vi "PicoScope5000aSetupStreaming.vi"(0 "error in":errorcluster, 1 "Device Info":T2, 2 "handle in":i16, 3 "Acquisition Settings":T3={"Auto Stop"=FALSE, "Desired Sample Interval"=4, "Pre-trigger Samples"=0, "Post-trigger Samples"=1000, "Down-Sample Ratio"=1, "Down-Sample Mode"=0, "Time Units"=2} {"Time Units" items=["Nanoseconds (ns)"=2, "Microseconds (us)"=3, "Milliseconds (ms)"=4, "Seconds (s)"=5]; "Down-Sample Mode" items=["None"=0, "Aggregate"=1, "Decimate"=2, "Average"=4]}, 4 "Buffer and Transfer Settings":T1={"startIndex"=0, "Samples"=1000000, "Down Sample Ratio"=1, "Down-Sample Mode"=0} {"Down-Sample Mode" items=["None"=0, "Aggregate"=1, "Decimate"=2, "Average"=4]; "Down Sample Ratio" step=1; "Samples" format="%_6p"}, 5 "enabled array":i16[](array[numeric]), 10 "Pointers In":u64[][](array[numeric])) -> (11 "Pointer array":u64[][](array[numeric]), 14 "error out":errorcluster, 16 "handle out":i16, 17 "Sample Interval":u32, 19 "sampleIntervalTimeUnits":u32)   [LabVIEW 2010]
doc: "Set up the data buffers and calls RunStreaming to start the device streaming.\nData will be copied from the driver buffers into the corresponding application buffers using the wrapper dll."
uses:
  ps5000a.dll
  ps5000aWrap.dll
panel:
  # "Overview Buffer Size is the size of the temporary buffers used to\nstore data before returning it to the application."
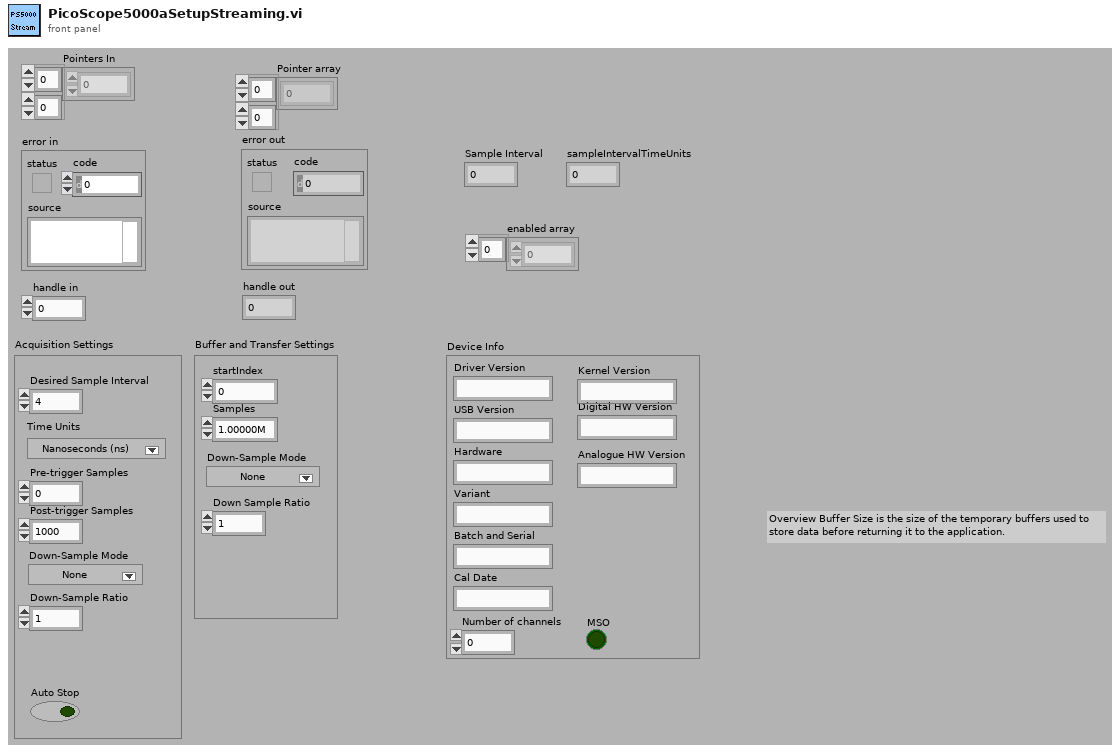
[diagram p1: front panel]
types:
  T1 = cluster{"startIndex":u64, "Samples":u64, "Down Sample Ratio":u64, "Down-Sample Mode":u32}
  T2 = cluster{"Driver Version":string, "USB Version":string, "Hardware":string, "Variant":string, "Batch and Serial":string, "Cal Date":string, "Kernel Version":string, "Digital HW Version":string, "Analogue HW Version":string, "MSO":bool, "Number of channels":i16}
  T3 = cluster{"Auto Stop":bool, "Desired Sample Interval":u32, "Pre-trigger Samples":u32, "Post-trigger Samples":u32, "Down-Sample Ratio":u32, "Down-Sample Mode":i32, "Time Units":u32}
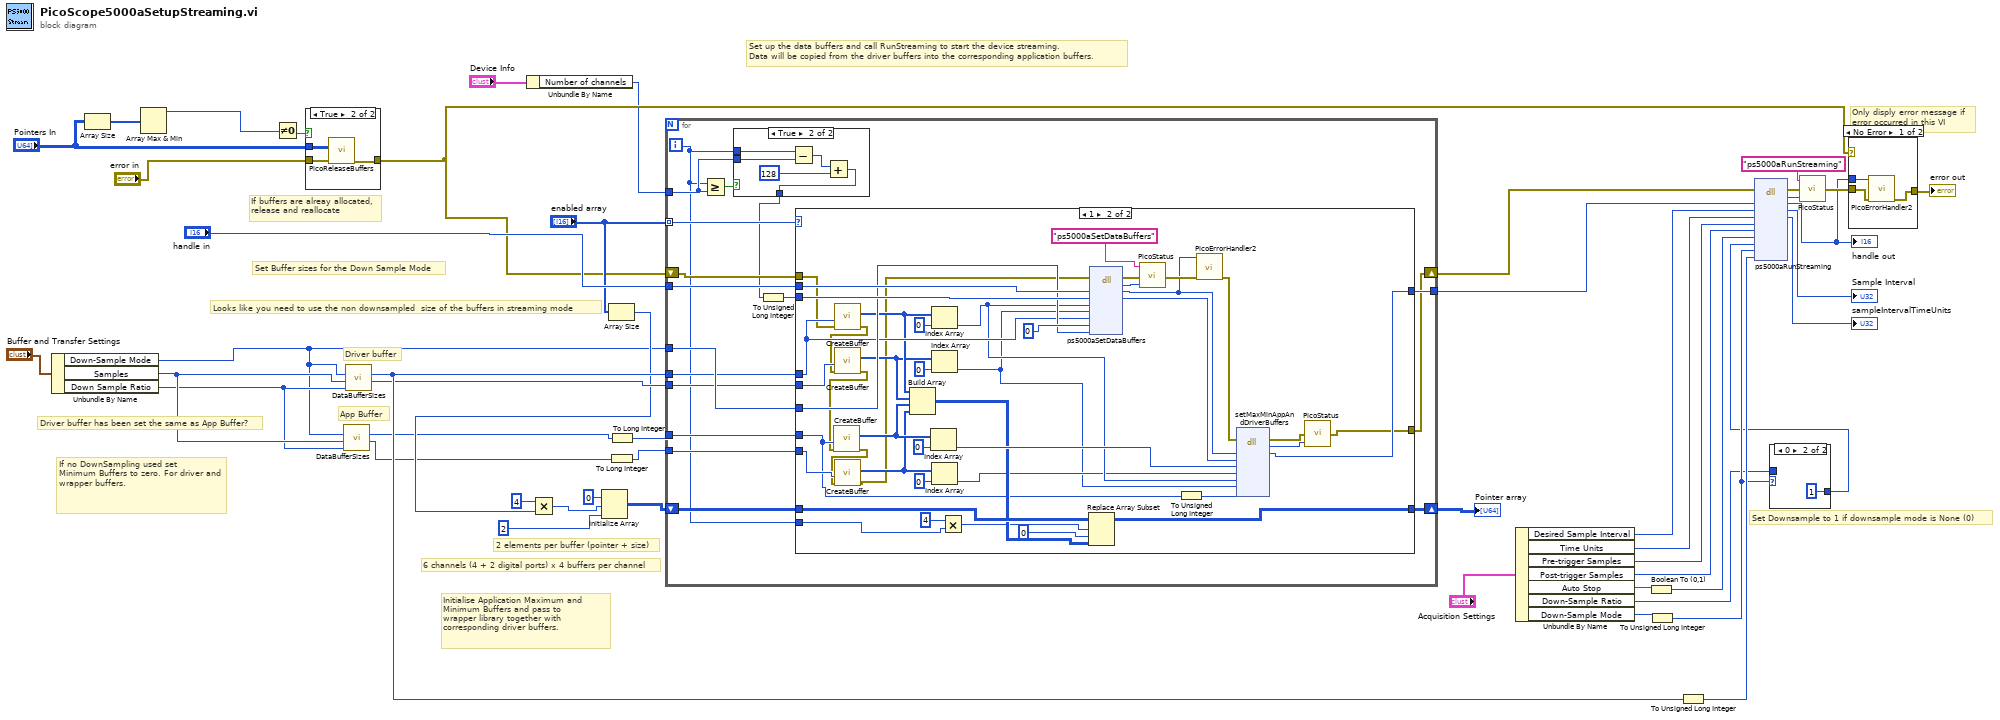
[diagram p0: block diagram]
diagram:
  # "Set Downsample to 1 if downsample mode is None (0)"
  # "Looks like you need to use the non downsampled  size of the buffers in streaming mode"
  # "If buffers are alreay allocated,\nrelease and reallocate"
  # "2 elements per buffer (pointer + size)"
  # "6 channels (4 + 2 digital ports) x 4 buffers per channel"
  # "App Buffer"
  # "Driver buffer"
  # "Driver buffer has been set the same as App Buffer?"
  # "Set Buffer sizes for the Down Sample Mode"
  # "If no DownSampling used set \nMinimum Buffers to zero. For driver and wrapper buffers."
  # "Initialise Application Maximum and\nMinimum Buffers and pass to \nwrapper library together with corresponding driver buffers."
  # "Only disply error message if\nerror occurred in this VI"
  # "Set up the data buffers and call RunStreaming to start the device streaming.\nData will be copied from the driver buffers into the corresponding application buffers."
  n1 = Unbundle By Name("Buffer and Transfer Settings") -> ("Down-Sample Mode"=w9:u32, "Samples"=w32:u64, "Down Sample Ratio"=w31:u64)
  n2 = Array Size(array="Pointers In") -> (size(s)=w12:i32[])
  n3 = Array Max & Min(array=w12) -> (max value=w11:i32)  [unwired: 3 out]
  n4 = Not Equal To 0?(x=w11) -> (x != 0?=w18:bool)
  n5 = case shown="True" w18 {
    tunnel: "Pointers In" -> [_ w51]
    tunnel: "error in" -> [w50 w52]
    tunnel: [w50 w53] -> w15
    frame False {
    }
    frame True {
      n6 = call "PicoReleaseBuffers.vi"("error in (no error)"=w52, "Pointer array"=w51) -> ("error out"=w53:errorcluster)  [unwired: 9 in]
    }
  }
  n7 = call "DataBufferSizes.vi"("Down Sample Ratio"=w31, "Number of Samples"=w32, "Down-Sample Mode"=w9) -> ("min Buffer Size"=w2:i32, "Max Buffer Size"=w3:i32)  [unwired: 7 in]
  n8 = call "DataBufferSizes.vi"("Down Sample Ratio"=w31, "Number of Samples"=w32, "Down-Sample Mode"=w9) -> ("min Buffer Size"=w29:i32, "Max Buffer Size"=w30:i32)  [unwired: 7 in]
  n9 = Unbundle By Name("Device Info") -> ("Number of channels"=w1:i16)
  n10 = Array Size(array="enabled array") -> (size(s)=w22:i32)
  n11 = Multiply(x=4, y=w22) -> (x*y=w23:i32)
  n12 = Initialize Array(u64 0 ("element"), w23, 2 ("dimension size")) -> (w13:u64[][])
  n13 = To Long Integer(number=w2) -> (32bit integer=w4:i32)
  n14 = To Long Integer(number=w3) -> (32bit integer=w5:i32)
  n15 = for {
    tunnel: "enabled array" -> [w62] mode=indexing
    tunnel: "handle in" -> [w70]
    tunnel: w9 -> [w69]
    tunnel: w5 -> [w68]
    tunnel: w30 -> [w67]
    tunnel: w29 -> [w66]
    tunnel: w4 -> [w65]
    tunnel: [w63] -> w25
    shift-right: [w61] -> w19
    shift-left: w15 -> [w60]
    shift-right: [w64] -> w28
    shift-left: w13 -> [w59]
    tunnel: w1 -> [w55]
    i -> [w54]
    n16 = Greater Or Equal?(x=w54, y=w55) -> (x >= y?=w57:bool)
    n17 = case shown="True" w57 {
      tunnel: [w71 w75] -> w56
      tunnel: w54 -> [w71 w73]
      tunnel: w55 -> [_ w72]
      frame False {
      }
      frame True {
        n18 = Subtract(x=w73, y=w72) -> (x-y=w74:i32)
        n19 = Add(x=w74, y=128) -> (x+y=w75:i32)
      }
    }
    n20 = To Unsigned Long Integer(number=w56) -> (unsigned 32bit integer=w58:u32)
    n21 = case shown="1" w62 {
      tunnel: w70 -> [w78 w123]
      tunnel: w60 -> [w77 w84]
      tunnel: w58 -> [_ w117]
      tunnel: w68 -> [_ w87]
      tunnel: w67 -> [_ w107]
      tunnel: w66 -> [_ w110]
      tunnel: w65 -> [_ w109]
      tunnel: w69 -> [_ w108]
      tunnel: w59 -> [w79 w101]
      tunnel: [w79 w100] -> w64
      tunnel: w54 -> [_ w97]
      tunnel: [w78 w93] -> w63
      tunnel: [w77 w92] -> w61
      frame 0, Default {
      }
      frame 1 {
        n22 = call "CreateBuffer.vi"("error in (no error)"=w84, "Buffer size"=w107) -> ("error out"=w83:errorcluster, "Pointer and BufferSize"=w105:u64[])  [unwired: 8 in]
        n23 = call "CreateBuffer.vi"("error in (no error)"=w83, "Buffer size"=w110) -> ("error out"=w82:errorcluster, "Pointer and BufferSize"=w104:u64[])  [unwired: 8 in]
        n24 = call "CreateBuffer.vi"("error in (no error)"=w82, "Buffer size"=w87) -> ("error out"=w81:errorcluster, "Pointer and BufferSize"=w103:u64[])  [unwired: 8 in]
        n25 = call "CreateBuffer.vi"("error in (no error)"=w81, "Buffer size"=w109) -> ("error out"=w80:errorcluster, "Pointer and BufferSize"=w102:u64[])  [unwired: 8 in]
        n26 = Build Array(w105, w104, w103, w102) -> (w96:u64[][])
        n27 = Index Array(array=w103, index=0) -> (element=w106:u64)
        n28 = Index Array(array=w105, index=0) -> (element=w99:u64)
        n29 = Index Array(array=w104, index=0) -> (element=w85:u64)
        n30 = Index Array(array=w102, index=0) -> (element=w86:u64)
        n31 = Multiply(x=4, y=w97) -> (x*y=w95:i32)
        n32 = Replace Array Subset(array=w101, new element=w96, index (row)=w95, index (col)=0 ("disabled index (row)")) -> (w100:u64[][])
        n33 = dll-call lib="ps5000a.dll" fn="ps5000aSetDataBuffers" ("ps3000.dll:_ps3000_open_unit@0")(error in=w80, "handle"=w123, "channel"=w117, "bufferMax"=w99, "bufferMin"=w85, "bufferLth"=w107, "segmentIndex"=u32 0, "downSampleRatioMode"=w108) -> (error out=w121:errorcluster, "PICO_STATUS"=w122:u32, "handle"=w89:i16, "channel"=w118:u32)  [unwired: 7 in, 1 out]
        n34 = call "PicoStatus.vi"("PICO STATUS"=w122, "error in"=w121, "source"="ps5000aSetDataBuffers") -> ("error out"=w91:errorcluster)
        n35 = To Unsigned Long Integer(number=w87) -> (unsigned 32bit integer=w88:u32)
        n36 = call "PicoErrorHandler2.vi"("error in (no error)"=w91, "handle In"=w89) -> ("error out"=w90:errorcluster)  [unwired: 9 in]
        n37 = dll-call lib="ps5000aWrap.dll" fn="setMaxMinAppAndDriverBuffers"(error in=w90, "handle"=w89, "channel"=w118, "appMaxBuffer"=w106, "appMinBuffer"=w86, "driverMaxBuffer"=w99, "driverMinBuffer"=w85, "bufferLength"=w88) -> (error out=w116:errorcluster, "PICO_STATUS"=w115:u32, "handle"=w93:i16)  [unwired: 8 in, 1 out]
        n38 = call "PicoStatus.vi"("PICO STATUS"=w115, "error in"=w116) -> ("error out"=w92:errorcluster)  [unwired: 1 in]
      }
    }
  }
  "Pointer array" <- w28
  n39 = Unbundle By Name("Acquisition Settings") -> ("Desired Sample Interval"=w42:u32, "Time Units"=w36:u32, "Pre-trigger Samples"=w41:u32, "Post-trigger Samples"=w40:u32, "Auto Stop"=w39:bool, "Down-Sample Ratio"=w7:u32, "Down-Sample Mode"=w37:i32)
  n40 = Boolean To (0,1)(Boolean=w39) -> (0, 1=w43:i16)
  n41 = To Unsigned Long Integer(number=w37) -> (unsigned 32bit integer=w8:u32)
  n42 = To Unsigned Long Integer(number=w30) -> (unsigned 32bit integer=w10:u32)
  n43 = case shown="0" w8 {
    tunnel: [w124 u32 1 ("Down-Sample Ratio")] -> w6
    tunnel: w7 -> [w124 _]
    frame Default {
    }
    frame 0 {
    }
  }
  n44 = dll-call lib="ps5000a.dll" fn="ps5000aRunStreaming" ("ps5000a.dll:_ps3000_open_unit@0")(error in=w19, "handle"=w25, "sampleInterval"=w42, "sampleIntervalTimeUnits"=w36, "maxPreTriggerSamples"=w41, "maxPostTriggerSamples"=w40, "autoStop"=w43, "downSampleRatio"=w6, "downSampleRatioMode"=w8, "overviewBufferSize"=w10) -> (error out=w47:errorcluster, "PICO_STATUS"=w48:u32, "handle"=w14:i16, "sampleInterval"=→"Sample Interval":u32, "sampleIntervalTimeUnits"=→"sampleIntervalTimeUnits":u32)  [unwired: 8 in, 1 out]
  "handle out" <- w14
  n45 = call "PicoStatus.vi"("PICO STATUS"=w48, "error in"=w47, "source"="ps5000aRunStreaming") -> ("error out"=w45:errorcluster)
  n46 = case shown="No Error" w15 {
    tunnel: [w127 w129] -> w49
    tunnel: w45 -> [w128 w129]
    tunnel: w14 -> [w126 _]
    frame No Error {
      n47 = call "PicoErrorHandler2.vi"("error in (no error)"=w128, "handle In"=w126) -> ("error out"=w127:errorcluster)  [unwired: 9 in]
    }
    frame Error {
    }
  }
  "error out" <- w49
